vi "FRC Wizard - Dashboard.vi"() -> ()   [LabVIEW 2025]
uses:
  <resource>/plugins/NewDialogFiles/ProjectWizards/ProjectWizard.llb/ProjectWizard Navigation Button States.ctl
  <resource>/plugins/NewDialogFiles/ProjectWizards/ProjectWizard.llb/ProjectWizard Navigation Button State.ctl
  <resource>/plugins/NewDialogFiles/ProjectWizards/ProjectWizard.llb/ProjectWizard Navigation Buttons.ctl
  <resource>/plugins/NewDialogFiles/ProjectWizards/FRC/frc project type.ctl
  <resource>/plugins/NewDialogFiles/ProjectWizards/FRC/FRC Strings.vi
panel:
  out "project folder flag":bool
  in  "Tab Control":enum32{"Page 1"}(tab)
  in  "Framework Choice":T1(radio)
  out "Picture-0":picture
  in  "Project folder":path
  in  "Project name":string
  in  "Shutdown user event":refnum<user-event>
  in  "Subpanel Path user event":refnum<user-event>
  in  "Window Title user event":refnum<user-event>
  in  "Navigation Button States user event":refnum<user-event>
  in  "Navigation Buttons user event":refnum<event-registration>
  # "Select project name and folder"
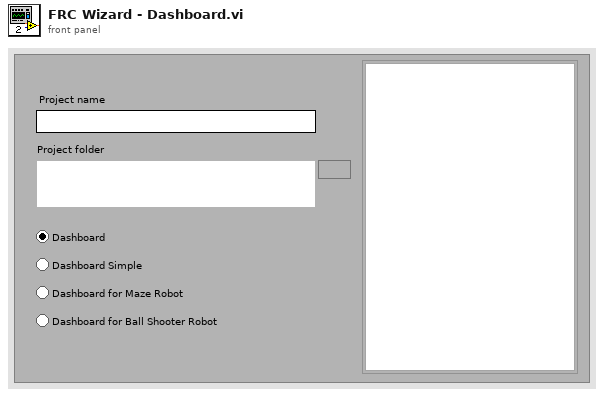
[diagram p1: front panel]
types:
  T1 = enum32{"dashboard", "dashboard simple", "dashboard maze", "dashboard shooter"}
  T2 = enum16{"Display", "Configure", "Hide Dialog", "Discard Ref"}
  T3 = typedef "ProjectWizard Navigation Button States.ctl" = T4[]
  T4 = typedef "ProjectWizard Navigation Button State.ctl" = cluster{"Navigation Button":T5, "Disabled":u8}
  T5 = typedef "ProjectWizard Navigation Buttons.ctl" = enum16{"Back", "Next", "Finish", "Cancel", "Help"}
  T6 = typedef "frc project type.ctl" = enum16{"arcade", "command control", "maze", "ball shooter", "dashboard", "dashboard simple", "dashboard maze", "dashboard shooter", "romi", "XRP"}
  T7 = typedef "RTNPA Navigation Buttons.ctl" = enum16{"Back", "Next", "Finish", "Cancel", "Help"}
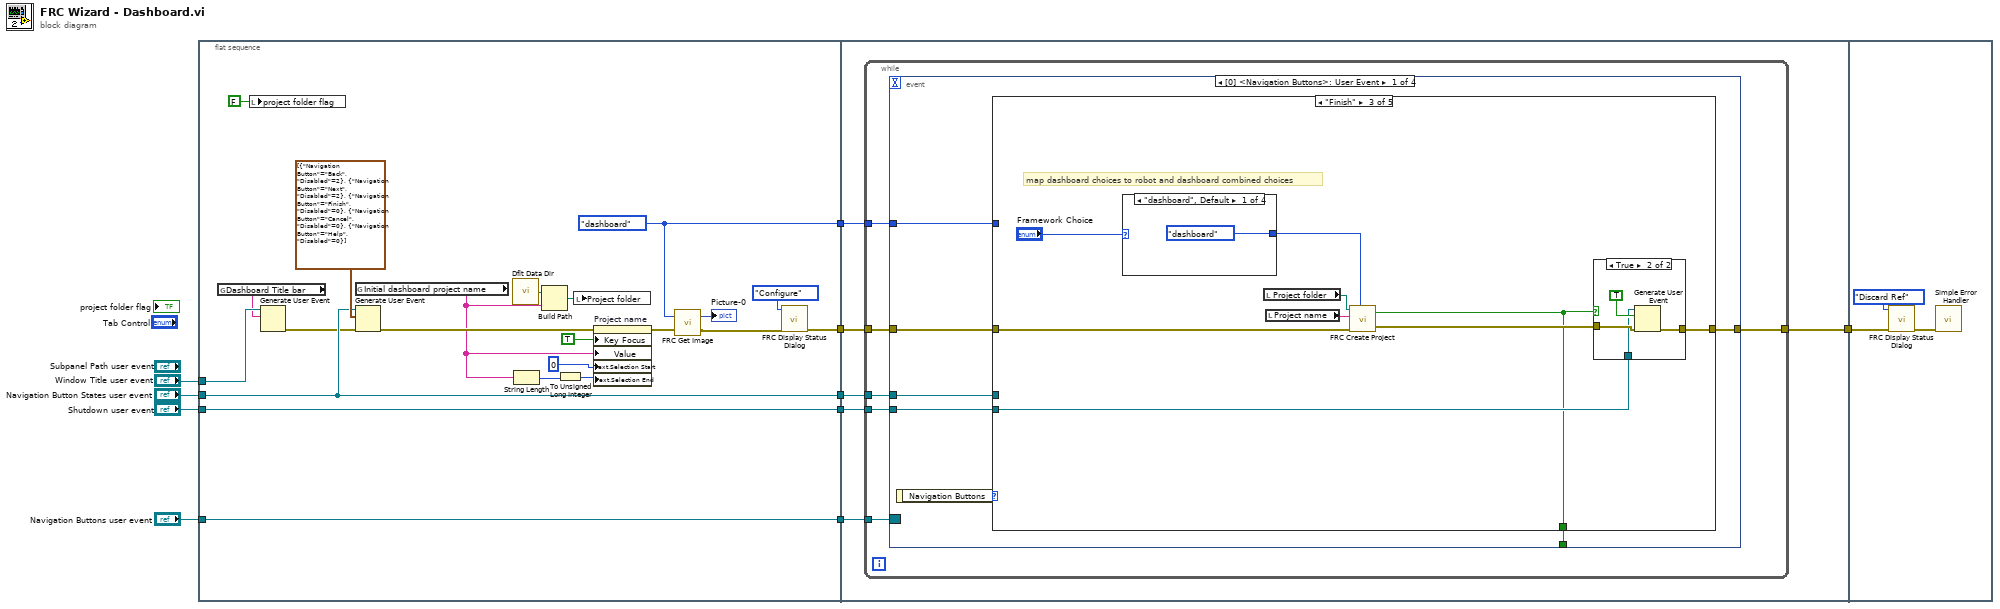
[diagram p0: block diagram]
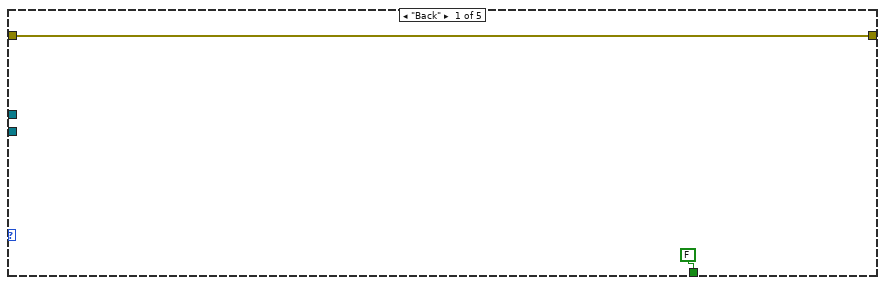
[diagram p2: hidden frame]
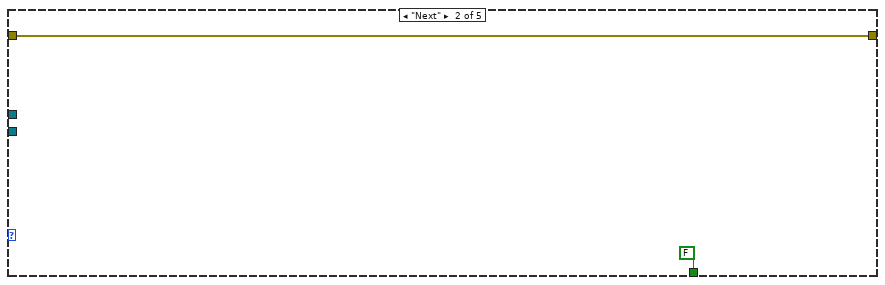
[diagram p3: hidden frame]
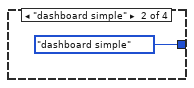
[diagram p4: hidden frame]
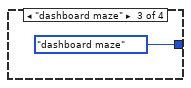
[diagram p5: hidden frame]
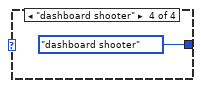
[diagram p6: hidden frame]
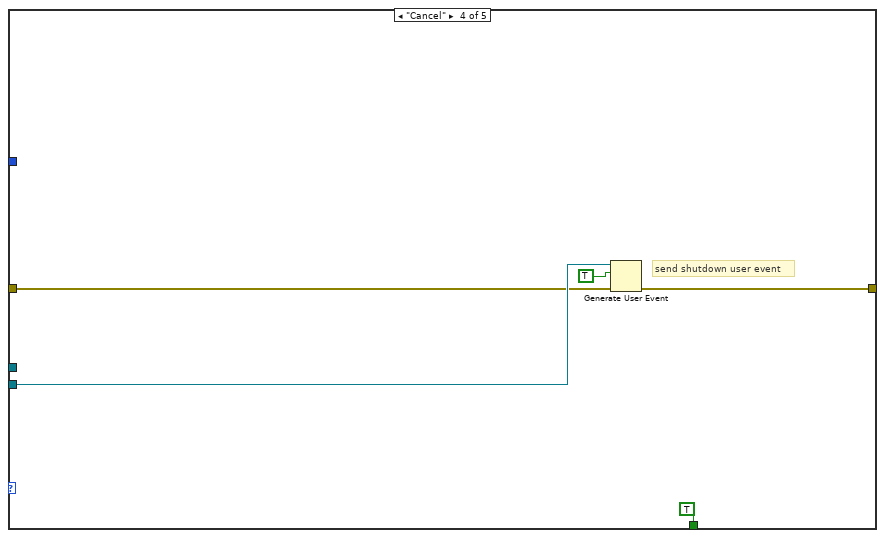
[diagram p8: hidden frame]
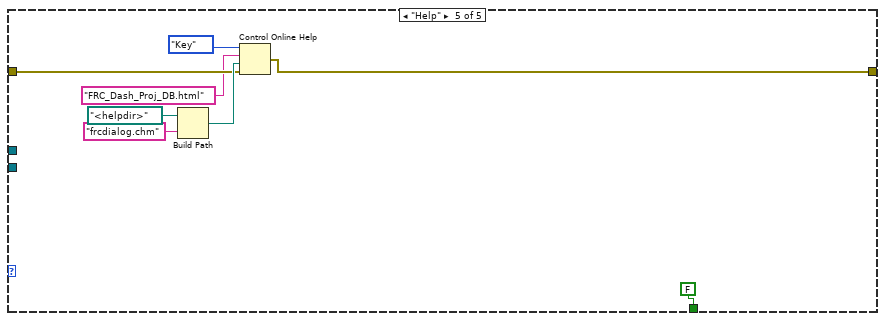
[diagram p9: hidden frame]
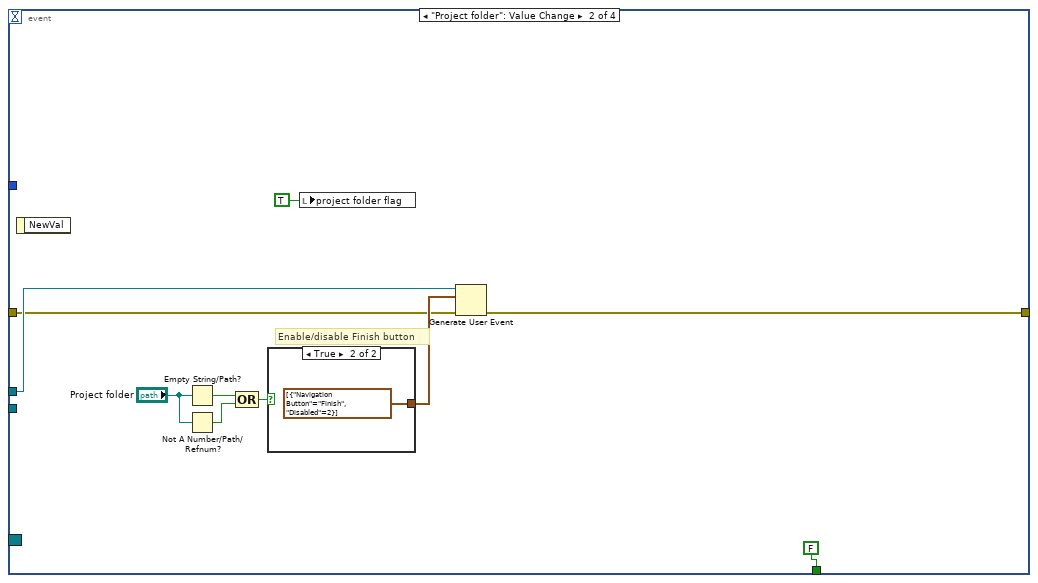
[diagram p10: hidden frame]
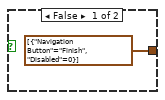
[diagram p11: hidden frame]
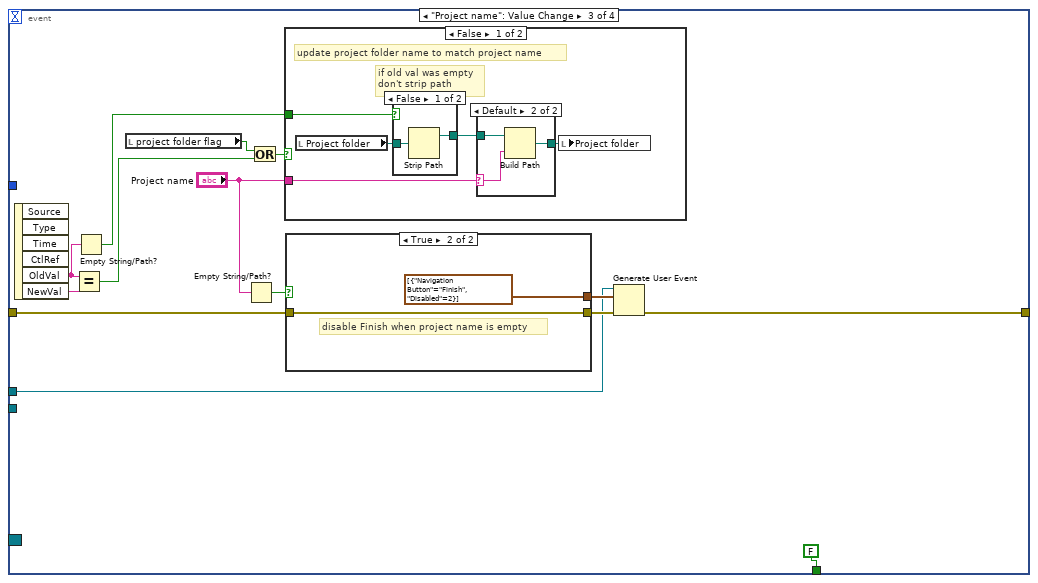
[diagram p12: hidden frame]
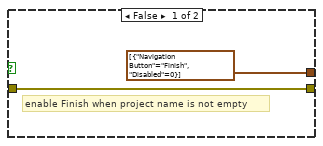
[diagram p16: hidden frame]
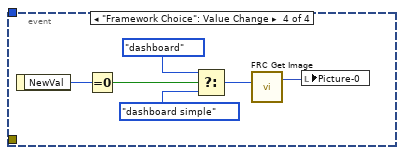
[diagram p17: hidden frame]
diagram:
  n1 = flat-sequence {
    tunnel: [w22] -> w6
    tunnel: [w32] -> w5
    tunnel: [w31] -> w4
    tunnel: [w18] -> w3
    tunnel: "Navigation Button States user event" -> [w22]
    tunnel: "Window Title user event" -> [w29]
    tunnel: "Navigation Buttons user event" -> [w32]
    tunnel: "Shutdown user event" -> [w31]
    tunnel: [w11] -> w1
    tunnel: w6 -> [w38]
    tunnel: w5 -> [w37]
    tunnel: w4 -> [w35]
    tunnel: w3 -> [w34]
    tunnel: [w36] -> w2
    tunnel: w1 -> [w33]
    tunnel: w2 -> [w137]
    frame #0 {
      w11 = frc_project_type."dashboard" ("frc project type")
      n2 = global read "FRC Strings.vi" "Dashboard Title bar"() -> (w26:string)
      n3 = local write "project folder flag"(FALSE ("project folder flag")) -> ()
      n4 = Generate User Event(user event=w29, event data cluster=w26) -> (error out=w21:errorcluster)  [unwired: 2 in, 1 out]
      n5 = global read "FRC Strings.vi" "Initial dashboard project name"() -> (w15:string)
      n6 = Generate User Event(user event=w22, event data cluster=T3 [{"Navigation Button"=enum."Back", "Disabled"=2}, {"Navigation Button"=enum."Next", "Disabled"=2}, {"Navigation Button"=enum."Finish", "Disabled"=0}, {"Navigation Button"=enum."Cancel", "Disabled"=0}, {"Navigation Button"=enum."Help", "Disabled"=0}] ("Navigation Button States"), error in=w21) -> (error out=w19:errorcluster)  [unwired: 1 in, 1 out]
      n7 = call <vilib>:"Dflt Data Dir.vi"() -> ("App:Default Data Directory"=w27:path)
      n8 = String Length(string=w15) -> (length=w23:i32)
      n9 = Build Path(base path=w27, name or relative path=w15) -> (appended path=w20:path)
      n10 = To Unsigned Long Integer(number=w23) -> (unsigned 32bit integer=w24:u32)
      n11 = local write "Project folder"(w20) -> ()
      n12 = property on="Project name" class="Str"(error in=w19, "Key Focus"=TRUE, "Value"=w15, "Text.Selection Start"=u32 0 ("Text.Selection:Start"), "Text.Selection End"=w24) -> (error out=w14:errorcluster)  [unwired: 1 in, 1 out]
      n13 = call <resource>:"FRC Get Image.vi"("error in"=w14, "frc project type"=w11) -> ("error out"=w13:errorcluster, "new picture"=→"Picture-0":picture)
      n14 = call <resource>:"FRC Display Status Dialog.vi"("error in"=w13, "Mode"=T2."Configure") -> ("error out"=w18:errorcluster)  [unwired: 2 in, 7 out]
    }
    frame #1 {
      n15 = while {
        tunnel: w37 -> [w45]
        tunnel: w38 -> [w44]
        tunnel: w34 -> [w43]
        tunnel: [w41] -> w36
        tunnel: w35 -> [w40]
        tunnel: w33 -> [w39]
        stop <- w42 stop-if-true
        n16 = event shown="[0] <Navigation Buttons>: User Event" {
          selector: w45 -> [_ _ _ _]
          dyn-events: _ -> [_ _ _ _]
          timeout: _ -> [_ _ _ _]
          tunnel: w44 -> [w48 w92 w107 _]
          tunnel: w43 -> [w50 w91 w112 _]
          tunnel: [w51 FALSE ("x = y?") FALSE ("x = y?") _] -> w42
          tunnel: [w49 w93 w109 _] -> w41
          tunnel: w40 -> [w47 _ _ _]
          tunnel: w39 -> [w46 _ _ _]
          event User Event {
            n17 = event-data() -> ("Navigation Buttons"=w52:T7)  [unwired: 1 out]
            n18 = case shown="\"Finish\"" w52 {
              tunnel: [FALSE ("x = y?") FALSE w59 TRUE FALSE] -> w51
              tunnel: w50 -> [w53 w55 w63 w75 w82]
              tunnel: [w53 w55 w65 w76 w83] -> w49
              tunnel: w48 -> [_ _ _ _ _]
              tunnel: w47 -> [_ _ w62 w77 _]
              tunnel: w46 -> [_ _ _ _ _]
              frame "Back" {
              }
              frame "Next" {
              }
              frame "Finish" {
                # "map dashboard choices to robot and dashboard combined choices"
                n19 = case shown="\"dashboard\", Default" "Framework Choice" {
                  tunnel: [frc_project_type."dashboard" ("frc project type") frc_project_type."dashboard simple" ("frc project type") frc_project_type."dashboard maze" ("frc project type") frc_project_type."dashboard shooter" ("frc project type")] -> w58
                  frame "dashboard", Default {
                  }
                  frame "dashboard simple" {
                  }
                  frame "dashboard maze" {
                  }
                  frame "dashboard shooter" {
                  }
                }
                n20 = local read "Project folder"() -> (w60:path)
                n21 = local read "Project name"() -> (w61:string)
                n22 = call <resource>:"FRC Create Project.vi"("Project folder"=w60, "Project name"=w61, "error in"=w63, "frc project type"=w58) -> ("proceed?"=w59:bool, "error out"=w64:errorcluster)  [unwired: 1 in]
                n23 = case shown="True" w59 {
                  tunnel: [w70 w74] -> w65
                  tunnel: w64 -> [w70 w72]
                  tunnel: w62 -> [_ w71]
                  frame False {
                  }
                  frame True {
                    n24 = Generate User Event(user event=w71, event data cluster=TRUE ("event data"), error in=w72) -> (error out=w74:errorcluster)  [unwired: 1 in, 1 out]
                  }
                }
              }
              frame "Cancel" {
                (unwired) refnum<k0> refnum
                # "send shutdown user event"
                n25 = Generate User Event(user event=w77, event data cluster=TRUE ("event data"), error in=w75) -> (error out=w76:errorcluster)  [unwired: 1 in, 1 out]
              }
              frame "Help" {
                n26 = Build Path(base path=path "<helpdir>", name or relative path="frcdialog.chm" ("CHM or HLP filename (lvdialog.chm)")) -> (appended path=w86:path)
                n27 = Control Online Help(1:w82, 2:w86, 3:"FRC_Dash_Proj_DB.html" ("String to search for"), 4:enum16{"Contents", "Key", "Close"}."Key" ("Operation")) -> (0:w83:errorcluster)
              }
            }
          }
          event "Project folder": Value Change {
            # "Enable/disable Finish button"
            n28 = event-data() -> ()  [unwired: 2 out]
            n29 = Empty String/Path?(string/path="Project folder") -> (empty?=w94:bool)
            n30 = Not A Number/Path/Refnum?(number/path/refnum="Project folder") -> (NaN/Path/Refnum?=w95:bool)
            n31 = Compound Arithmetic op=OR(w94, w95) -> (w96:bool)
            n32 = case shown="True" w96 {
              tunnel: [T3 [{"Navigation Button"=enum."Finish", "Disabled"=0}] ("Navigation Button States") T3 [{"Navigation Button"=enum."Finish", "Disabled"=2}] ("Navigation Button States")] -> w97
              frame False {
              }
              frame True {
              }
            }
            n33 = local write "project folder flag"(TRUE ("project folder flag")) -> ()
            n34 = Generate User Event(user event=w92, event data cluster=w97, error in=w91) -> (error out=w93:errorcluster)  [unwired: 1 in, 1 out]
          }
          event "Project name": Value Change {
            n35 = event-data() -> ("OldVal"=w101:string, "NewVal"=w105:string)  [unwired: 5 out]
            n36 = Equal?(x=w101, y=w105) -> (x = y?=w102:bool)
            n37 = Empty String/Path?(string/path=w101) -> (empty?=w100:bool)
            n38 = local read "project folder flag"() -> (w104:bool)
            n39 = Empty String/Path?(string/path="Project name") -> (empty?=w111:bool)
            n40 = Or(x=w104, y=w102) -> (x .or. y?=w103:bool)
            n41 = case shown="False" w103 {
              tunnel: "Project name" -> [w116 _]
              tunnel: w100 -> [w114 _]
              frame False {
                # "update project folder name to match project name"
                # "if old val was empty\ndon't strip path"
                n42 = local read "Project folder"() -> (w115:path)
                n43 = case shown="False" w114 {
                  tunnel: [w120 w121] -> w117
                  tunnel: w115 -> [w119 w121]
                  frame False {
                    n44 = Strip Path(path=w119) -> (stripped path=w120:path)  [unwired: 1 out]
                  }
                  frame True {
                  }
                }
                n45 = case shown="Default" w116 {
                  selector: w116 -> [_ w123]
                  tunnel: [w122 w125] -> w118
                  tunnel: w117 -> [w122 w124]
                  frame "" {
                  }
                  frame Default {
                    n46 = Build Path(base path=w124, name or relative path=w123) -> (appended path=w125:path)
                  }
                }
                n47 = local write "Project folder"(w118) -> ()
              }
              frame True {
                # "don't update project folder, user modified it manually\nor value didn't really change"
              }
            }
            n48 = case shown="True" w111 {
              tunnel: w112 -> [w126 w128]
              tunnel: [w126 w128] -> w110
              tunnel: [T3 [{"Navigation Button"=enum."Finish", "Disabled"=0}] ("Navigation Button States") T3 [{"Navigation Button"=enum."Finish", "Disabled"=2}] ("Navigation Button States")] -> w108
              frame False {
                # "enable Finish when project name is not empty"
              }
              frame True {
                # "disable Finish when project name is empty"
              }
            }
            n49 = Generate User Event(user event=w107, event data cluster=w108, error in=w110) -> (error out=w109:errorcluster)  [unwired: 1 in, 1 out]
          }
          event "Framework Choice": Value Change {
            n50 = event-data() -> ("NewVal"=w135:T1)  [unwired: 1 out]
            n51 = Equal To 0?(x=w135) -> (x = 0?=w132:bool)
            n52 = Select(t=frc_project_type."dashboard" ("frc project type"), s=w132, f=frc_project_type."dashboard simple" ("frc project type")) -> (s? t:f=w131:T6)
            n53 = call <resource>:"FRC Get Image.vi"("frc project type"=w131) -> ("new picture"=w130:picture)  [unwired: 1 in, 1 out]
            n54 = local write "Picture-0"(w130) -> ()
          }
        }
      }
    }
    frame #2 {
      n55 = call <resource>:"FRC Display Status Dialog.vi"("error in"=w137, "Mode"=T2."Discard Ref") -> ("error out"=w136:errorcluster)  [unwired: 2 in, 7 out]
      n56 = call <vilib>:"Simple Error Handler.vi"("error in (no error)"=w136) -> ()  [unwired: 1 in, 8 out]
    }
  }
